vi "JsonRpcResponseClusterToString.vi"(8 "error in (no error)":errorcluster, 10 "JsonRPCHttpResponseBody":T1) -> (0 "error out":errorcluster, 2 "JsonRPCHttpResonseBodyString":string)   [LabVIEW 2017]
uses:
  <vilib>/LVH/i3 JSON/JSON Generation/Create Value Files/Create Value - Object.vi
  <vilib>/LVH/i3 JSON/JSON Generation/Add Object Parameter Files/Add Object Parameter - String.vi
  <vilib>/LVH/i3 JSON/JSON Generation/Add Object Parameter Files/Add Object Parameter - Object.vi
  <vilib>/LVH/i3 JSON/JSON Generation/Add Object Parameter Files/Add Object Parameter - Numeric.vi
  <vilib>/LVH/i3 JSON/i3-json.lvlib
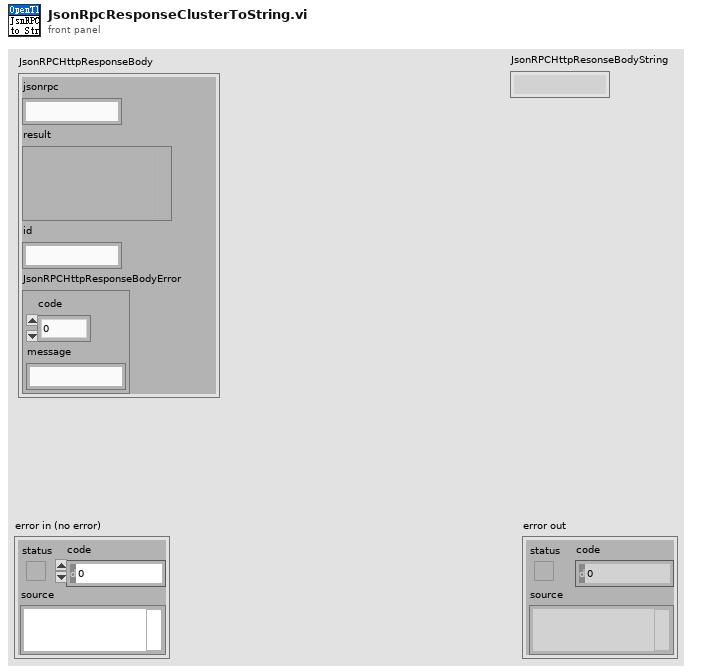
[diagram p1: front panel]
types:
  T1 = cluster{"jsonrpc":string, "result":variant, "id":string, "JsonRPCHttpResponseBodyError":cluster{"code":i32, "message":string}}
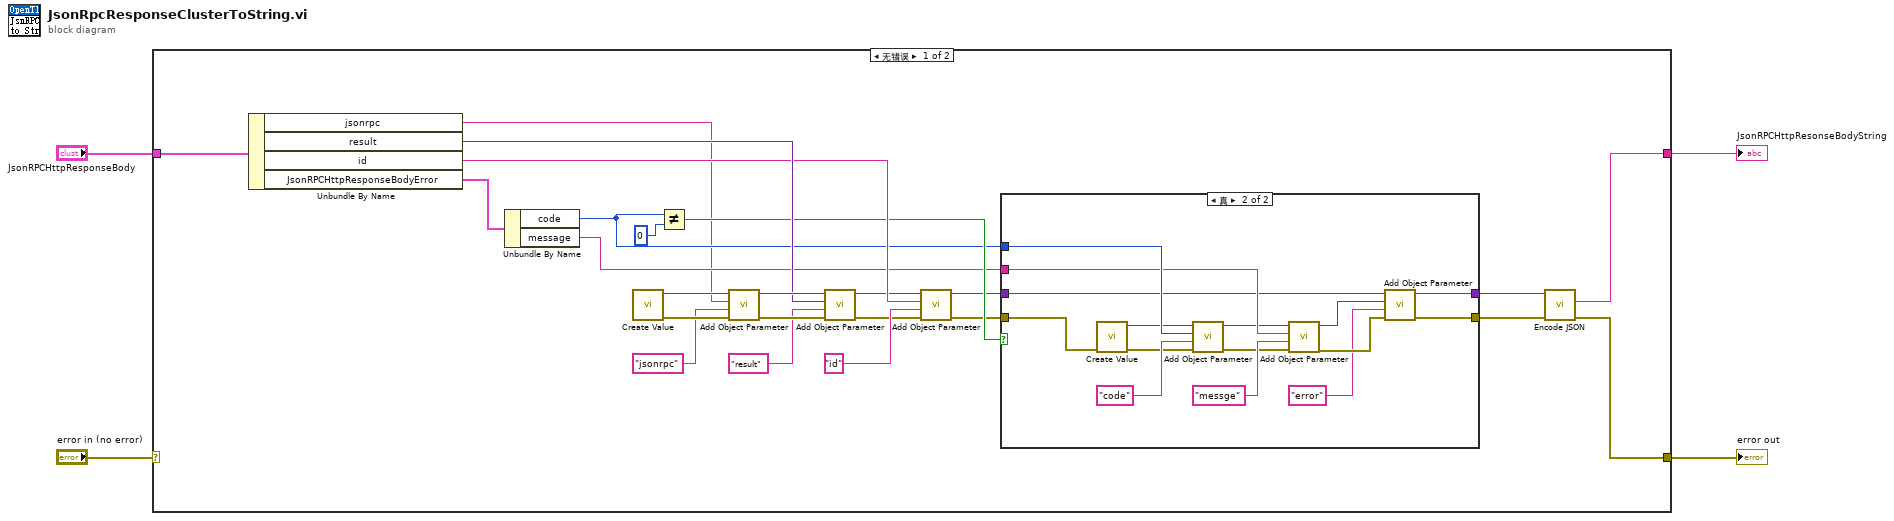
[diagram p0: block diagram]
diagram:
  n1 = case shown="无错误" "error in (no error)" {
    selector: "error in (no error)" -> [_ w46]
    tunnel: [w25 w46] -> w3
    tunnel: "JsonRPCHttpResponseBody" -> [w28 _]
    tunnel: [w26 _] -> w1
    frame No Error {
      n2 = Unbundle By Name(w28) -> ("jsonrpc"=w6:string, "result"=w19:variant, "id"=w17:string, "JsonRPCHttpResponseBodyError"=w27:cluster{"code":i32, "message":string})
      n3 = Unbundle By Name(w27) -> ("code"=w8:i32, "message"=w7:string)
      n4 = call-poly <vilib>:"Create Value.vi"() -> ("error out"=w23:errorcluster, "JSON Tree"=w24:variant)  [unwired: 10 in]
      n5 = Not Equal?(x=w8, y=0) -> (x != y?=w13:bool)
      n6 = call-poly <vilib>:"Add Object Parameter.vi"("error in (no error)"=w23, "Name"="jsonrpc" ("String"), "String"=w6, "JSON Tree in (JSON Object)"=w24) -> ("error out"=w21:errorcluster, "JSON Tree out (JSON Object)"=w22:variant)  [unwired: 6 in]
      n7 = call-poly <vilib>:"Add Object Parameter.vi"("error in (no error)"=w21, "Name"="result" ("String"), "JSON Object"=w19, "JSON Tree in (JSON Object)"=w22) -> ("error out"=w15:errorcluster, "JSON Tree out (JSON Object)"=w16:variant)  [unwired: 6 in]
      n8 = call-poly <vilib>:"Add Object Parameter.vi"("error in (no error)"=w15, "Name"="id" ("String"), "String"=w17, "JSON Tree in (JSON Object)"=w16) -> ("error out"=w10:errorcluster, "JSON Tree out (JSON Object)"=w12:variant)  [unwired: 6 in]
      n9 = case shown="真" w13 {
        tunnel: w12 -> [w30 w36]
        tunnel: [w30 w32] -> w11
        tunnel: w10 -> [w29 w39]
        tunnel: [w29 w33] -> w9
        tunnel: w8 -> [_ w45]
        tunnel: w7 -> [_ w41]
        frame False {
        }
        frame True {
          n10 = call-poly <vilib>:"Create Value.vi"("error in (no error)"=w39) -> ("error out"=w40:errorcluster, "JSON Tree"=w38:variant)  [unwired: 9 in]
          n11 = call-poly <vilib>:"Add Object Parameter.vi"("error in (no error)"=w40, "Name"="code" ("String"), "Numeric"=w45, "JSON Tree in (JSON Object)"=w38) -> ("error out"=w42:errorcluster, "JSON Tree out (JSON Object)"=w37:variant)  [unwired: 6 in]
          n12 = call-poly <vilib>:"Add Object Parameter.vi"("error in (no error)"=w42, "Name"="messge" ("String"), "String"=w41, "JSON Tree in (JSON Object)"=w37) -> ("error out"=w34:errorcluster, "JSON Tree out (JSON Object)"=w35:variant)  [unwired: 6 in]
          n13 = call-poly <vilib>:"Add Object Parameter.vi"("error in (no error)"=w34, "Name"="error" ("String"), "JSON Object"=w35, "JSON Tree in (JSON Object)"=w36) -> ("error out"=w33:errorcluster, "JSON Tree out (JSON Object)"=w32:variant)  [unwired: 6 in]
        }
      }
      n14 = call <vilib>:"Encode JSON.vi"("error in (no error)"=w9, "JSON Tree"=w11) -> ("error out"=w25:errorcluster, "String"=w26:string)  [unwired: 4 in]
    }
    frame Error {
    }
  }
  "error out" <- w3
  "JsonRPCHttpResonseBodyString" <- w1
